vi "Move_Ground.vi"(0 "State":T1={"Tick"=0, "Phase"=0, "PhaseTicks"=0, "Level"=1, "Room"=0, "X10"=0, "Y10"=0, "VY10"=0, "Mode"=0, "Facing"=0, "Run"=0, "Vert"=0, "StandY"=0, "EntryX10"=0, "EntryY10"=0, "EntryMode"=0, "Lives"=4, "Score"=0, "NextLife"=10000, "KeyR"=0, "KeyB"=0, "KeyY"=0, "Torch"=FALSE, "FloorPhase"=0, "Dead"=FALSE, "LevelStart"=FALSE, "Quit"=FALSE, "Sound"=0, "Seed"=12345, "DemoStep"=0, "Tiles"=[], "World"=[], "Enemies"=[], "Highscores"=[], "Name"=[0, 0, 0], "Cursor"=0}, 5 "Jump":bool, 7 "XA10":i32, 11 "error in":errorcluster) -> (4 "Mode":i32, 6 "X10":i32, 8 "Y10":i32, 10 "VY10":i32, 15 "error out":errorcluster)   [LabVIEW 2020, in "GH_Engine.lvlib"]
doc: "Claude on the ground, one tick: stands on a wall, thin floor or ladder top; jump; step onto a ladder or rope (Up/Down); grab a pole over its hole; otherwise fall (Mode 2). Inline subVI of Player_Move."
uses:
  GH_Engine.lvlib
  Level/GH_Level.lvlib
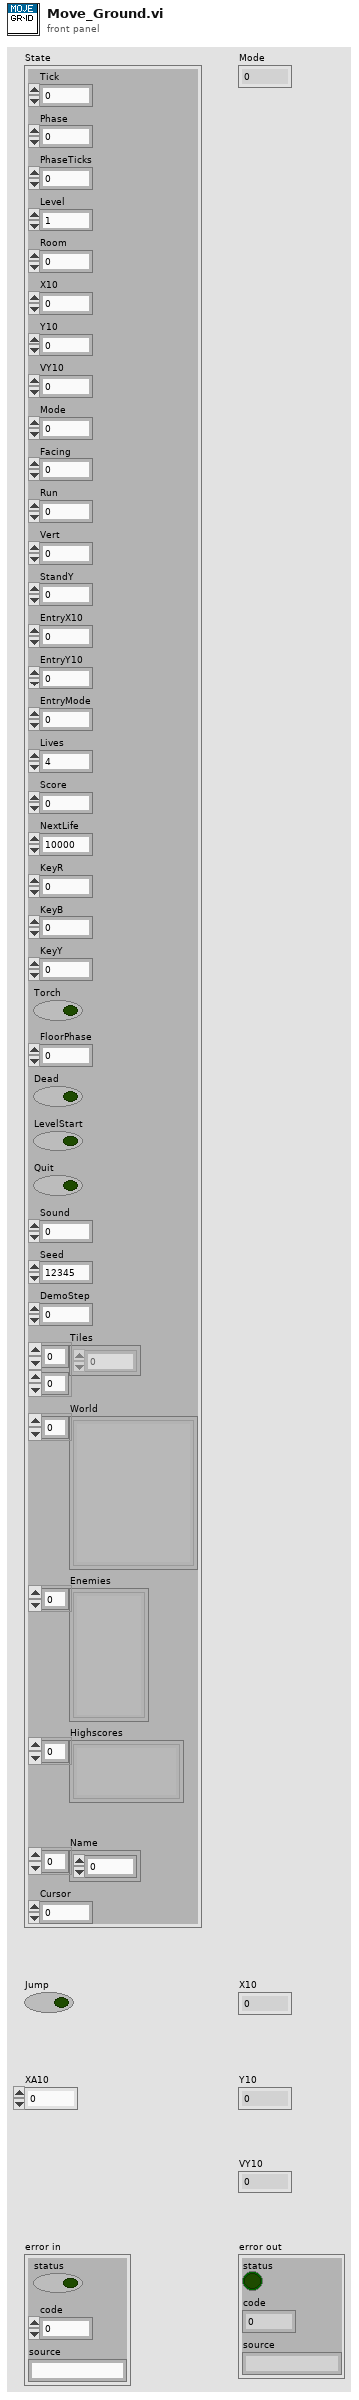
[diagram p1: front panel]
types:
  T1 = cluster{"Tick":u32, "Phase":i32, "PhaseTicks":i32, "Level":i32, "Room":i32, "X10":i32, "Y10":i32, "VY10":i32, "Mode":i32, "Facing":i32, "Run":i32, "Vert":i32, "StandY":i32, "EntryX10":i32, "EntryY10":i32, "EntryMode":i32, "Lives":i32, "Score":i32, "NextLife":i32, "KeyR":i32, "KeyB":i32, "KeyY":i32, "Torch":bool, "FloorPhase":i32, "Dead":bool, "LevelStart":bool, "Quit":bool, "Sound":i32, "Seed":u32, "DemoStep":i32, "Tiles":u8[][], "World":cluster{"ID":string, "Depth":i32, "Column":i32, "Tiles":u8[][]}[], "Enemies":cluster{"Kind":i32, "X10":i32, "Y10":i32, "Dir":i32, "Mode":i32}[], "Highscores":cluster{"Score":i32, "Name":string}[], "Name":i32[], "Cursor":i32}
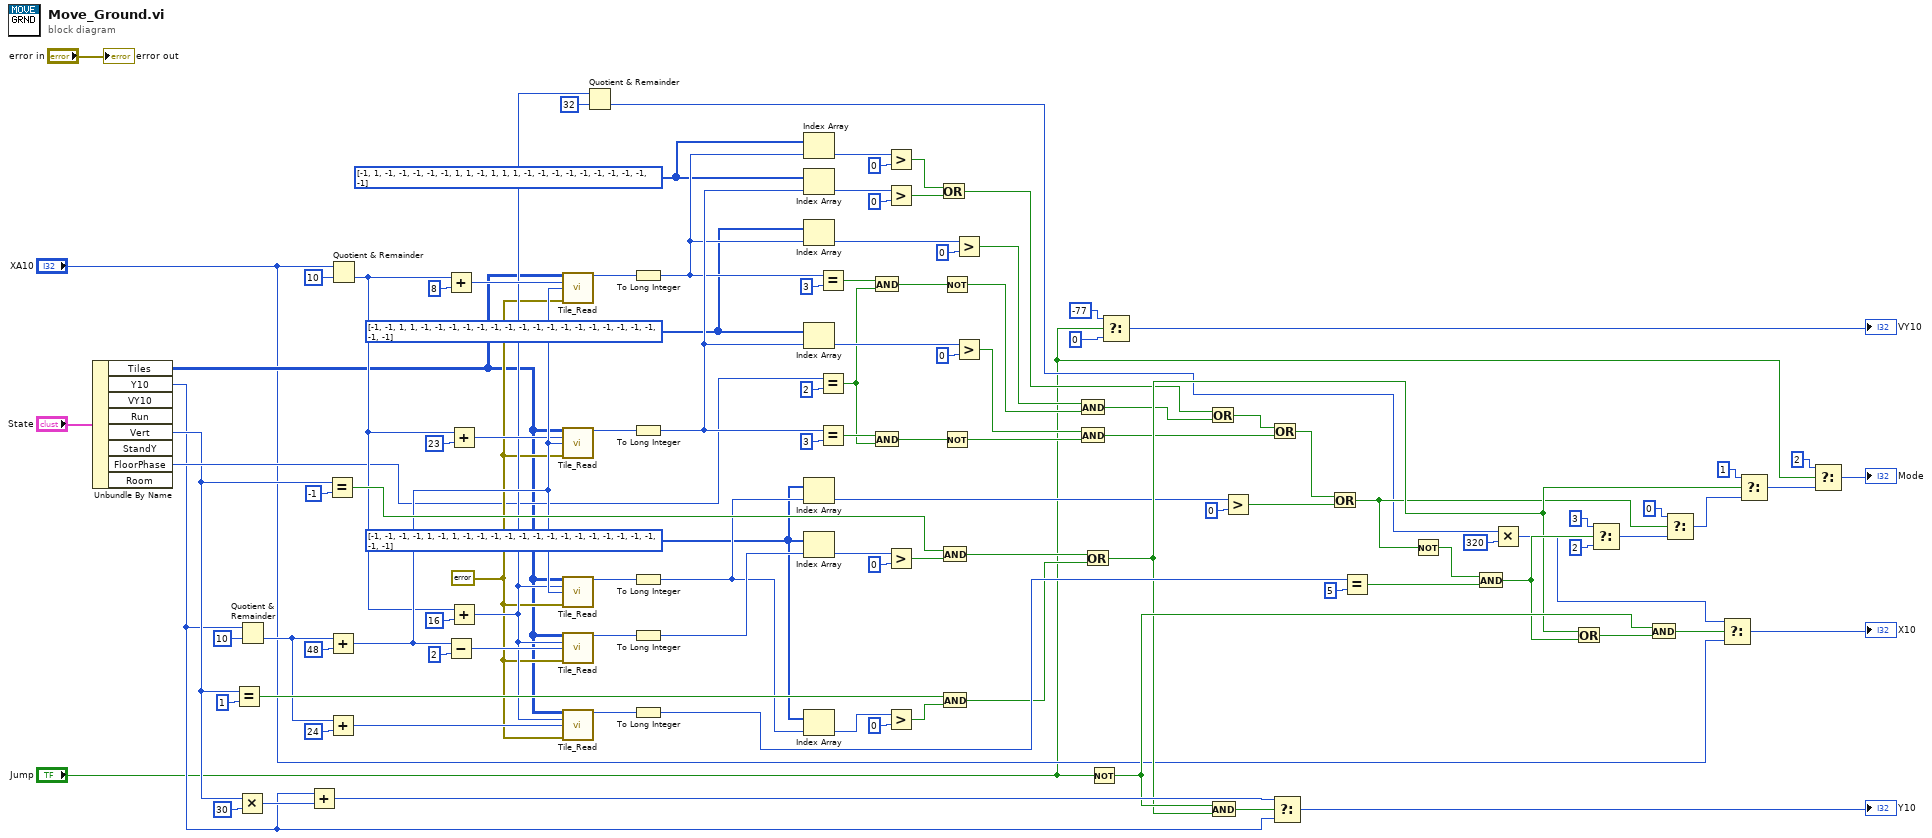
[diagram p0: block diagram]
diagram:
  w14 = errorcluster {"status"=FALSE, "code"=0, "source"=""} ("no error")
  w11 = i32[] [-1, -1, -1, -1, 1, -1, 1, -1, -1, -1, -1, -1, -1, -1, -1, -1, -1, -1, -1, -1, -1, -1, -1] ("Ladder or rope")
  w10 = i32[] [-1, -1, 1, 1, -1, -1, -1, -1, -1, -1, -1, -1, -1, -1, -1, -1, -1, -1, -1, -1, -1, -1, -1] ("Thin floor")
  w9 = i32[] [-1, 1, -1, -1, -1, -1, -1, 1, 1, -1, 1, 1, 1, -1, -1, -1, -1, -1, -1, -1, -1, -1, -1] ("Solid")
  n1 = Unbundle By Name("State") -> ("Tiles"=w5:u8[][], "Y10"=w6:i32, "Vert"=w7:i32, "FloorPhase"=w8:i32)  [unwired: 4 out]
  n2 = Equal?(x=w7, y=1) -> (x = y?=w77:bool)
  n3 = Multiply(x=w7, y=30) -> (x*y=w106:i32)
  n4 = Quotient & Remainder(x=w6, y=10) -> (floor(x/y)=w24:i32)  [unwired: 1 out]
  n5 = Add(x=w6, y=w106) -> (x+y=w107:i32)
  n6 = Equal?(x=w7, y=-1) -> (x = y?=w67:bool)
  n7 = Add(x=w24, y=48) -> (x+y=w26:i32)
  n8 = Add(x=w24, y=24) -> (x+y=w85:i32)
  n9 = Quotient & Remainder(x="XA10", y=10) -> (floor(x/y)=w16:i32)  [unwired: 1 out]
  n10 = Add(x=w16, y=8) -> (x+y=w20:i32)
  n11 = Subtract(x=w26, y=2) -> (x-y=w69:i32)
  n12 = Add(x=w16, y=23) -> (x+y=w22:i32)
  n13 = Add(x=w16, y=16) -> (x+y=w18:i32)
  n14 = call "Tile_Read.vi"("Tiles"=w5, "X"=w20, "Y"=w26, "error in"=w14) -> ("Tile"=w31:u8)  [unwired: 10 in, 1 out]
  n15 = call "Tile_Read.vi"("Tiles"=w5, "X"=w22, "Y"=w26, "error in"=w14) -> ("Tile"=w33:u8)  [unwired: 10 in, 1 out]
  n16 = call "Tile_Read.vi"("Tiles"=w5, "X"=w18, "Y"=w26, "error in"=w14) -> ("Tile"=w35:u8)  [unwired: 10 in, 1 out]
  n17 = call "Tile_Read.vi"("Tiles"=w5, "X"=w18, "Y"=w69, "error in"=w14) -> ("Tile"=w70:u8)  [unwired: 10 in, 1 out]
  n18 = call "Tile_Read.vi"("Tiles"=w5, "X"=w18, "Y"=w85, "error in"=w14) -> ("Tile"=w86:u8)  [unwired: 10 in, 1 out]
  n19 = Quotient & Remainder(x=w18, y=32) -> (floor(x/y)=w28:i32)  [unwired: 1 out]
  n20 = To Long Integer(number=w31) -> (32bit integer=w32:i32)
  n21 = To Long Integer(number=w33) -> (32bit integer=w34:i32)
  n22 = To Long Integer(number=w35) -> (32bit integer=w36:i32)
  n23 = To Long Integer(number=w70) -> (32bit integer=w71:i32)
  n24 = To Long Integer(number=w86) -> (32bit integer=w87:i32)
  n25 = Index Array(array=w9, index=w32) -> (element=w37:i32)
  n26 = Index Array(array=w9, index=w34) -> (element=w40:i32)
  n27 = Index Array(array=w10, index=w32) -> (element=w43:i32)
  n28 = Index Array(array=w10, index=w34) -> (element=w51:i32)
  n29 = Index Array(array=w11, index=w36) -> (element=w59:i32)
  n30 = Index Array(array=w11, index=w71) -> (element=w72:i32)
  n31 = Index Array(array=w11, index=w36) -> (element=w78:i32)
  n32 = Equal?(x=w32, y=3) -> (x = y?=w47:bool)
  n33 = Equal?(x=w8, y=2) -> (x = y?=w13:bool)
  n34 = Equal?(x=w34, y=3) -> (x = y?=w55:bool)
  n35 = And(x=w47, y=w13) -> (x .and. y?=w48:bool)
  n36 = And(x=w55, y=w13) -> (x .and. y?=w56:bool)
  n37 = Greater?(x=w37, y=0) -> (0:w39:bool)
  n38 = Greater?(x=w40, y=0) -> (0:w42:bool)
  n39 = Greater?(x=w72, y=0) -> (0:w74:bool)
  n40 = Greater?(x=w78, y=0) -> (0:w80:bool)
  n41 = Or(x=w39, y=w42) -> (x .or. y?=w62:bool)
  n42 = And(x=w67, y=w74) -> (x .and. y?=w75:bool)
  n43 = And(x=w77, y=w80) -> (x .and. y?=w81:bool)
  n44 = Not(x=w48) -> (.not. x?=w49:bool)
  n45 = Not(x=w56) -> (.not. x?=w57:bool)
  n46 = Greater?(x=w43, y=0) -> (0:w45:bool)
  n47 = Greater?(x=w51, y=0) -> (0:w53:bool)
  n48 = And(x=w45, y=w49) -> (x .and. y?=w50:bool)
  n49 = And(x=w53, y=w57) -> (x .and. y?=w58:bool)
  n50 = Or(x=w75, y=w81) -> (x .or. y?=w82:bool)
  n51 = Not(x="Jump") -> (.not. x?=w91:bool)
  n52 = Select(t=-77, s="Jump", f=0) -> (s? t:f=→"VY10":i32)
  n53 = Or(x=w62, y=w50) -> (x .or. y?=w63:bool)
  n54 = And(x=w91, y=w82) -> (x .and. y?=w104:bool)
  n55 = Greater?(x=w59, y=0) -> (0:w61:bool)
  n56 = Or(x=w63, y=w58) -> (x .or. y?=w64:bool)
  n57 = Select(t=w107, s=w104, f=w6) -> (s? t:f=→"Y10":i32)
  n58 = Or(x=w64, y=w61) -> (x .or. y?=w65:bool)
  n59 = Equal?(x=w87, y=5) -> (x = y?=w89:bool)
  n60 = Not(x=w65) -> (.not. x?=w83:bool)
  n61 = And(x=w83, y=w89) -> (x .and. y?=w90:bool)
  n62 = Multiply(x=w28, y=320) -> (x*y=w30:i32)
  n63 = Or(x=w82, y=w90) -> (x .or. y?=w101:bool)
  n64 = Select(t=3, s=w90, f=2) -> (s? t:f=w97:i32)
  n65 = And(x=w91, y=w101) -> (x .and. y?=w102:bool)
  n66 = Select(t=0, s=w65, f=w97) -> (s? t:f=w98:i32)
  n67 = Select(t=w30, s=w102, f="XA10") -> (s? t:f=→"X10":i32)
  n68 = Select(t=1, s=w82, f=w98) -> (s? t:f=w99:i32)
  n69 = Select(t=2, s="Jump", f=w99) -> (s? t:f=→"Mode":i32)
  "error out" <- "error in"
